vi "Pi Microseconds.vi"(8 "error in (no error)":errorcluster) -> (0 "error out":errorcluster, 3 "us":u64=1000)   [LabVIEW 2020, in "wiringPi.lvlib"]
doc: "<b>_______________________________________________________________</b>\n** Author: Juan José Villacorta\n** LabVIEW wrapper for C library <b> wiringPi </b>,\n** https://github.com/WiringPi/WiringPi\n<b>_______________________________________________________________</b>\n\n/*\n * piMicros64:\n * Return a number of microseconds as an unsigned int64.\n *********************************************************************************\n */"
uses:
  wiringPi.lvlib
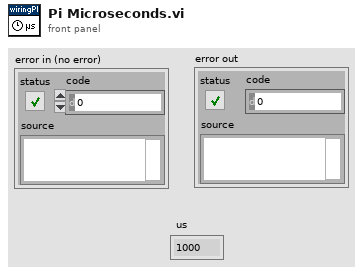
[diagram p1: front panel]
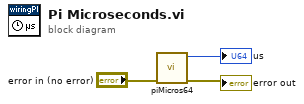
[diagram p0: block diagram]
diagram:
  n1 = call "piMicros64.vi"("error in (no error)"="error in (no error)") -> ("error out"=→"error out":errorcluster, "us"=→"us":u64)  [unwired: 9 in]
